vi "MotionProfileControlData.vi"() -> ()   [LabVIEW 2017]
uses:
  General/MotionProfiling/TypeDefs/ArmMotionProfileControl.ctl
  General/MotionProfiling/TypeDefs/TrajectoryPoint.ctl
  <vilib>/Rock Robotics/WPI/ThirdParty/Phoenix-LabVIEW/Motor Controller/Controls/CTRE_Phoenix_MotorControl_TrajectoryPointTimeDur.ctl
  General/MotionProfiling/TypeDefs/DriveMotionProfileControl.ctl
  Pathfinder/Pathfinder-LabVIEW/Pathfinder-Lib/VIs/Segment.ctl
  Pathfinder/Pathfinder-LabVIEW/Pathfinder-Lib/Pathfinder.lvlib
panel:
  in  "RightDriveMPControl":T1
  in  "LeftDriveMPControl":T1
  in  "ArmRotateMPControl":T4 {"Trajectory Points"."Time (ms)" items=["TrajectoryDuration_0ms"=0, "TrajectoryDuration_5ms"=5, "TrajectoryDuration_10ms"=10, "TrajectoryDuration_20ms"=20, "TrajectoryDuration_30ms"=30, "TrajectoryDuration_40ms"=40, "TrajectoryDuration_50ms"=50, "TrajectoryDuration_100ms"=100]}
  in  "ArmExtendMPControl":T4 {"Trajectory Points"."Time (ms)" items=["TrajectoryDuration_0ms"=0, "TrajectoryDuration_5ms"=5, "TrajectoryDuration_10ms"=10, "TrajectoryDuration_20ms"=20, "TrajectoryDuration_30ms"=30, "TrajectoryDuration_40ms"=40, "TrajectoryDuration_50ms"=50, "TrajectoryDuration_100ms"=100]}
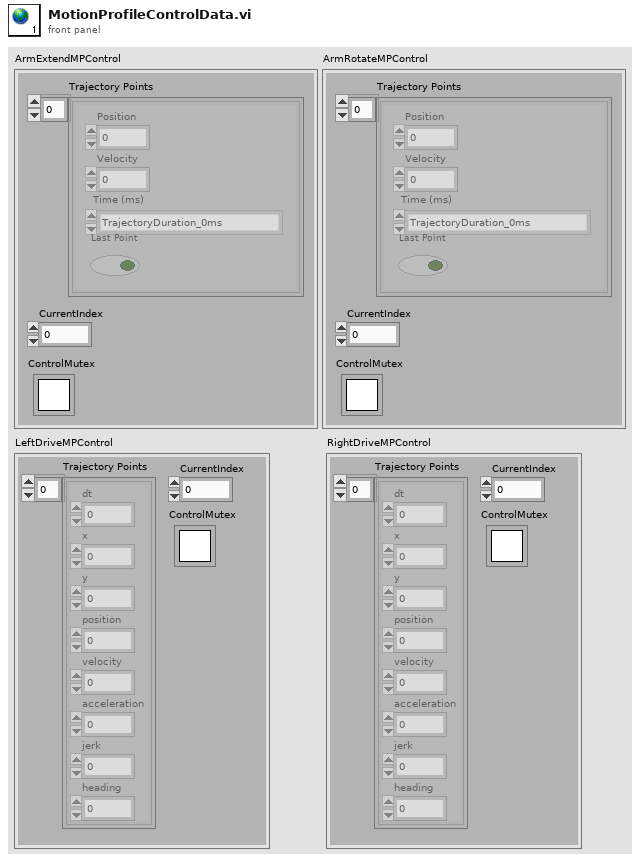
[diagram p1: front panel]
types:
  T1 = typedef "DriveMotionProfileControl.ctl" = cluster{"ControlMutex":T2, "Trajectory Points":T3[], "CurrentIndex":u32}
  T2 = typedef "Semaphore RefNum" = refnum<k1>
  T3 = typedef "Pathfinder.lvlib/Segment.ctl" = cluster{"dt":dbl, "x":dbl, "y":dbl, "position":dbl, "velocity":dbl, "acceleration":dbl, "jerk":dbl, "heading":dbl}
  T4 = typedef "ArmMotionProfileControl.ctl" = cluster{"ControlMutex":T2, "Trajectory Points":T5[], "CurrentIndex":u32}
  T5 = typedef "TrajectoryPoint.ctl" = cluster{"Position ":dbl, "Velocity ":dbl, "Time (ms)":T6, "Last Point":bool}
  T6 = typedef "CTRE_Phoenix_MotorControl_TrajectoryPointTimeDur.ctl" = i32
diagram:
